vi "Test MQTT-3.1.3-5.vi"(8 "error in (no error)":errorcluster, 11 "Connection Config":refnum<class "Connection.lvclass">) -> (0 "error out":errorcluster, 3 "Connection Config dup":refnum<class "Connection.lvclass">)   [LabVIEW 2013]
uses:
  <vilib>/LabVIEW Open Source Project/MQTT Connection/MQTT_Connection/Connection/Connection.lvclass
  <vilib>/LabVIEW Open Source Project/MQTT Control Packets/Control Packets/CONNACK/Connect Return Code -- enum.ctl
  <vilib>/addons/_JKI Toolkits/Caraya/classes/Test/Test.lvclass
  <vilib>/LabVIEW Open Source Project/MQTT Control Packets/Control Packets/CONNACK/CONNACK.lvclass
  <vilib>/addons/_JKI Toolkits/Caraya/classes/Assert/Assert.lvclass
  <vilib>/LabVIEW Open Source Project/MQTT Client/Client class/Client.lvclass
  <vilib>/LabVIEW Open Source Project/MQTT Connection/MQTT_Base/Base Class/MQTT_Base.lvclass
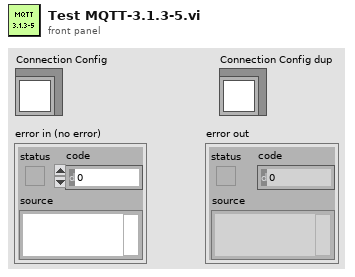
[diagram p1: front panel]
types:
  T1 = typedef "MQTT_Control_Packets.lvlib/CONNACK.lvclass/Connect Return Code -- enum.ctl" = enum16{"Connection accepted", "Unacceptable protocol version", "Identifier Rejected", "Server Unavailable", "Bad Username or Password", "Not Authorized"}
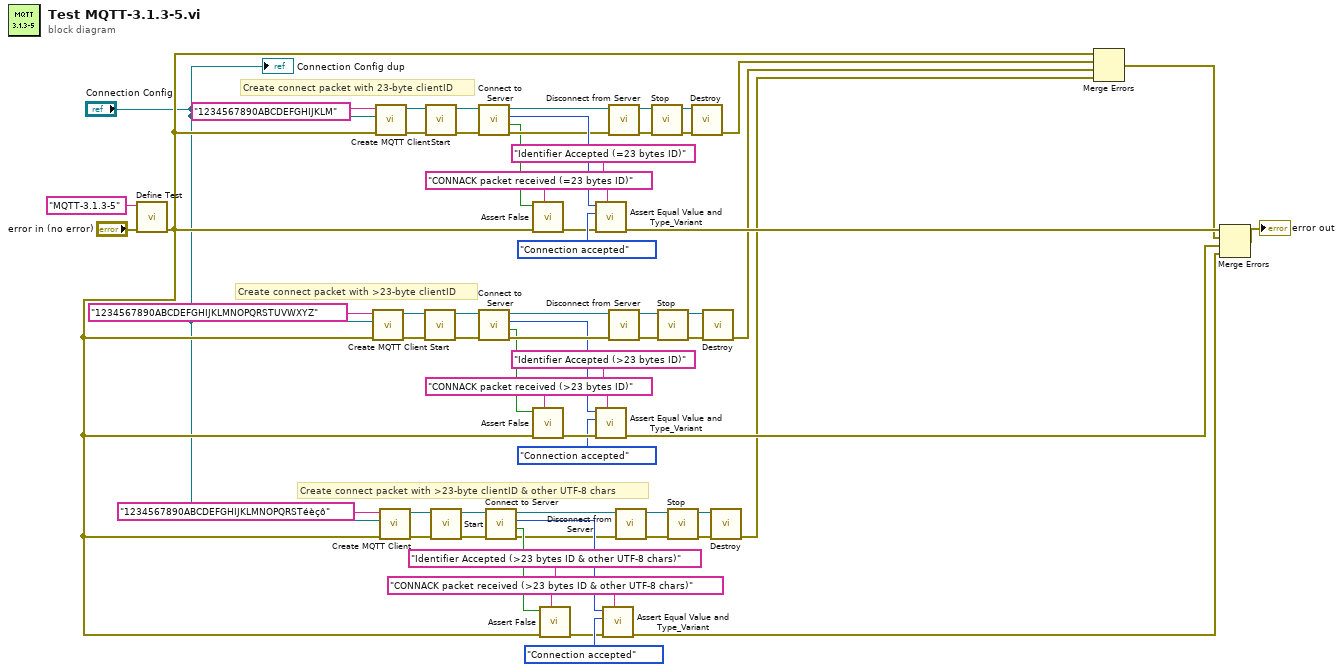
[diagram p0: block diagram]
diagram:
  # "Create connect packet with >23-byte clientID & other UTF-8 chars"
  # "Create connect packet with >23-byte clientID"
  # "Create connect packet with 23-byte clientID"
  n1 = call <vilib>:"Define Test.vi"("error in (no error)"="error in (no error)", "Label (VI Title)"="MQTT-3.1.3-5") -> ("error out"=w31:errorcluster)  [unwired: 9 in]
  n2 = call <vilib>:"Create MQTT Client.vi"("error in (no error)"=w31, "Connection Configuration"="Connection Config", "ID (empty:generate new)"="1234567890ABCDEFGHIJKLMNOPQRSTUVWXYZ" ("Client ID (empty: generate new)")) -> ("error out"=w14:errorcluster, "Client out"=w16:refnum<class "Client.lvclass">)  [unwired: 7 in]
  n3 = call <vilib>:"Create MQTT Client.vi"("error in (no error)"=w31, "Connection Configuration"="Connection Config", "ID (empty:generate new)"="1234567890ABCDEFGHIJKLM" ("Client ID (empty: generate new)")) -> ("error out"=w22:errorcluster, "Client out"=w24:refnum<class "Client.lvclass">)  [unwired: 7 in]
  n4 = call <vilib>:"Create MQTT Client.vi"("error in (no error)"=w31, "Connection Configuration"="Connection Config", "ID (empty:generate new)"="1234567890ABCDEFGHIJKLMNOPQRSTéèçô" ("Client ID (empty: generate new)")) -> ("error out"=w8:errorcluster, "Client out"=w7:refnum<class "Client.lvclass">)  [unwired: 7 in]
  n5 = call <vilib>:"Start.vi"("error in (no error)"=w14, "MQTT_Base in"=w16) -> ("error out"=w13:errorcluster, "MQTT_Base out"=w15:refnum<class "Client.lvclass">)  [unwired: 7 in, 1 out]
  n6 = call <vilib>:"Start.vi"("error in (no error)"=w22, "MQTT_Base in"=w24) -> ("error out"=w21:errorcluster, "MQTT_Base out"=w23:refnum<class "Client.lvclass">)  [unwired: 7 in, 1 out]
  n7 = call <vilib>:"Start.vi"("error in (no error)"=w8, "MQTT_Base in"=w7) -> ("error out"=w5:errorcluster, "MQTT_Base out"=w6:refnum<class "Client.lvclass">)  [unwired: 7 in, 1 out]
  n8 = call <vilib>:"Connect to Server.vi"("error in (no error)"=w21, "Client in"=w23) -> ("error out"=w51:errorcluster, "timed out"=w50:bool, "Return Code"=w53:T1, "Client out"=w52:refnum<class "Client.lvclass">)  [unwired: 6 in]
  n9 = call <vilib>:"Connect to Server.vi"("error in (no error)"=w13, "Client in"=w15) -> ("error out"=w49:errorcluster, "timed out"=w40:bool, "Return Code"=w41:T1, "Client out"=w48:refnum<class "Client.lvclass">)  [unwired: 6 in]
  n10 = call <vilib>:"Connect to Server.vi"("error in (no error)"=w5, "Client in"=w6) -> ("error out"=w32:errorcluster, "timed out"=w39:bool, "Return Code"=w38:T1, "Client out"=w33:refnum<class "Client.lvclass">)  [unwired: 6 in]
  n11 = call <vilib>:"Assert False.vi"("Label"="CONNACK packet received (=23 bytes ID)", "error in (no error)"=w31, "False?"=w50) -> ("error out"=w57:errorcluster)  [unwired: 8 in]
  n12 = call <vilib>:"Assert False.vi"("Label"="CONNACK packet received (>23 bytes ID)", "error in (no error)"=w31, "False?"=w40) -> ("error out"=w45:errorcluster)  [unwired: 8 in]
  n13 = call <vilib>:"Assert False.vi"("Label"="CONNACK packet received (>23 bytes ID & other UTF-8 chars)", "error in (no error)"=w31, "False?"=w39) -> ("error out"=w35:errorcluster)  [unwired: 8 in]
  n14 = call <vilib>:"Assert Equal Value and Type_Variant.vi"("Label"="Identifier Accepted (=23 bytes ID)", "error in (no error)"=w57, "Y"=Connect_Return_Code_--_enum."Connection accepted" ("Return Code"), "X"=w53) -> ("error out"=w62:errorcluster)  [unwired: 7 in]
  n15 = call <vilib>:"Assert Equal Value and Type_Variant.vi"("Label"="Identifier Accepted (>23 bytes ID)", "error in (no error)"=w45, "Y"=Connect_Return_Code_--_enum."Connection accepted" ("Return Code"), "X"=w41) -> ("error out"=w42:errorcluster)  [unwired: 7 in]
  n16 = call <vilib>:"Assert Equal Value and Type_Variant.vi"("Label"="Identifier Accepted (>23 bytes ID & other UTF-8 chars)", "error in (no error)"=w35, "Y"=Connect_Return_Code_--_enum."Connection accepted" ("Return Code"), "X"=w38) -> ("error out"=w29:errorcluster)  [unwired: 7 in]
  n17 = call <vilib>:"Disconnect from Server.vi"("error in (no error)"=w51, "Client in"=w52) -> ("error out"=w20:errorcluster, "Client out"=w18:refnum<class "Client.lvclass">)  [unwired: 7 in, 1 out]
  n18 = call <vilib>:"Disconnect from Server.vi"("error in (no error)"=w49, "Client in"=w48) -> ("error out"=w9:errorcluster, "Client out"=w10:refnum<class "Client.lvclass">)  [unwired: 7 in, 1 out]
  n19 = call <vilib>:"Disconnect from Server.vi"("error in (no error)"=w32, "Client in"=w33) -> ("error out"=w1:errorcluster, "Client out"=w3:refnum<class "Client.lvclass">)  [unwired: 7 in, 1 out]
  n20 = call <vilib>:"Stop.vi"("error in (no error)"=w20, "MQTT_Base in"=w18) -> ("error out"=w19:errorcluster, "MQTT_Base out"=w17:refnum<class "Client.lvclass">)  [unwired: 7 in, 1 out]
  n21 = call <vilib>:"Stop.vi"("error in (no error)"=w9, "MQTT_Base in"=w10) -> ("error out"=w12:errorcluster, "MQTT_Base out"=w11:refnum<class "Client.lvclass">)  [unwired: 7 in, 1 out]
  n22 = call <vilib>:"Stop.vi"("error in (no error)"=w1, "MQTT_Base in"=w3) -> ("error out"=w4:errorcluster, "MQTT_Base out"=w2:refnum<class "Client.lvclass">)  [unwired: 7 in, 1 out]
  n23 = call <vilib>:"Destroy.vi"("error in (no error)"=w19, "MQTT_Base in"=w17) -> ("error out"=w26:errorcluster)  [unwired: 8 in, 1 out]
  n24 = call <vilib>:"Destroy.vi"("error in (no error)"=w12, "MQTT_Base in"=w11) -> ("error out"=w27:errorcluster)  [unwired: 8 in, 1 out]
  n25 = call <vilib>:"Destroy.vi"("error in (no error)"=w4, "MQTT_Base in"=w2) -> ("error out"=w28:errorcluster)  [unwired: 8 in, 1 out]
  n26 = Merge Errors(w31, w26, w27, w28) -> (w55:errorcluster)
  n27 = Merge Errors(w62, w55, w42, w29) -> (→"error out":errorcluster)
  "Connection Config dup" <- "Connection Config"
